vi "Write Outputs.vi"(8 "error in (no error)":errorcluster, 10 "Analog Outputs":sgl[](array[numeric]), 11 "An Out in":refnum<class "An Out I2C.lvclass">) -> (0 "error out":errorcluster, 3 "An Out out":refnum<class "An Out I2C.lvclass">)   [LabVIEW 2020, in "CTI-Peripheral.lvlib" / "An Out I2C.lvclass"]
uses:
  An Out I2C.lvclass
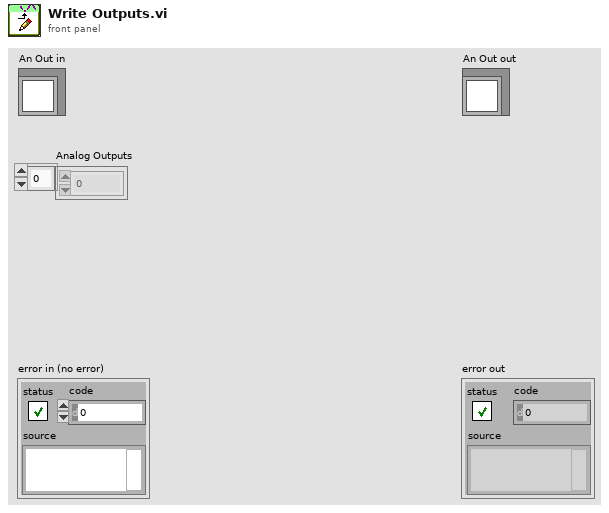
[diagram p1: front panel]
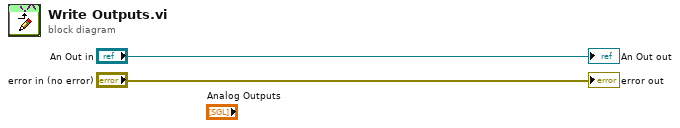
[diagram p0: block diagram]
diagram:
  "error out" <- "error in (no error)"
  "An Out out" <- "An Out in"
